vi "Lock-in_dem_mul Multiple Inputs and Outputs.vi"(3 "Phase&Tc":T1(array[cluster])=[{"Phase"=-4.587448254233148, "Time constant"=0.10000000000000009, "Set TimeConstant"=FALSE, "Autophase"=FALSE, "Order"=2.0}, {"Phase"=0.0, "Time constant"=0.2, "Set TimeConstant"=FALSE, "Autophase"=FALSE, "Order"=2.0}, {"Phase"=0.0, "Time constant"=0.0, "Set TimeConstant"=FALSE, "Autophase"=FALSE, "Order"=0.0}, {"Phase"=0.0, "Time constant"=0.0, "Set TimeConstant"=FALSE, "Autophase"=FALSE, "Order"=0.0}] {"Phase" min=0.0 max=360.0 scale=0.0..360.0}, 4 "Ref in":T2(array[cluster])=[{"Ref X"=array[40000 elements], "Ref Y"=array[40000 elements], "AI Rate"=200000.0, "AI Block Size"=40000.0, "Frequency"=20.0, "Ref amp"=5.0}, {"Ref X"=array[40000 elements], "Ref Y"=array[40000 elements], "AI Rate"=200000.0, "AI Block Size"=40000.0, "Frequency"=20.0, "Ref amp"=5.0}, {"Ref X"=array[40000 elements], "Ref Y"=array[40000 elements], "AI Rate"=200000.0, "AI Block Size"=40000.0, "Frequency"=20.0, "Ref amp"=5.0}, {"Ref X"=array[40000 elements], "Ref Y"=array[40000 elements], "AI Rate"=200000.0, "AI Block Size"=40000.0, "Frequency"=20.0, "Ref amp"=5.0}] {"Ref amp" step=0.001 format="%0.4f"; "Frequency" step=0.001 format="%0.4f"; "AI Block Size" step=0.001 format="%0.4f"; "AI Rate" step=0.001 format="%0.4f"}, 5 "Signal":dbl[][](array[numeric])=array4x40000[160000 elements]) -> (1 "Demodulation":dbl[][](array[numeric])=[[0.032308985716257205, -0.0020089800684537727, 0.032371384878394444, -3.5583001590229886], [0.023385861272623584, -0.0014539178662531169, 0.02343101330770514, -3.5574201885889787], [-3.111140914765216e-05, 2.7289487058700542e-06, 3.123206852318323e-05, -5.0131650508604935], [-3.1370210865590166e-05, 3.1631661467659442e-06, 3.1532606636697875e-05, -5.751181571584788]])   [LabVIEW 2013]
uses:
  <vilib>/Analysis/3filter.llb/Filter Passband Type.ctl
  <vilib>/Analysis/baseanly.llb/Mean (DBL).vi
  <vilib>/ptbypt/NI_PtbyPt.lvlib
  <vilib>/Analysis/NI_AALBase.lvlib
panel:
  out "Waveform Chart":dbl[][](graph)
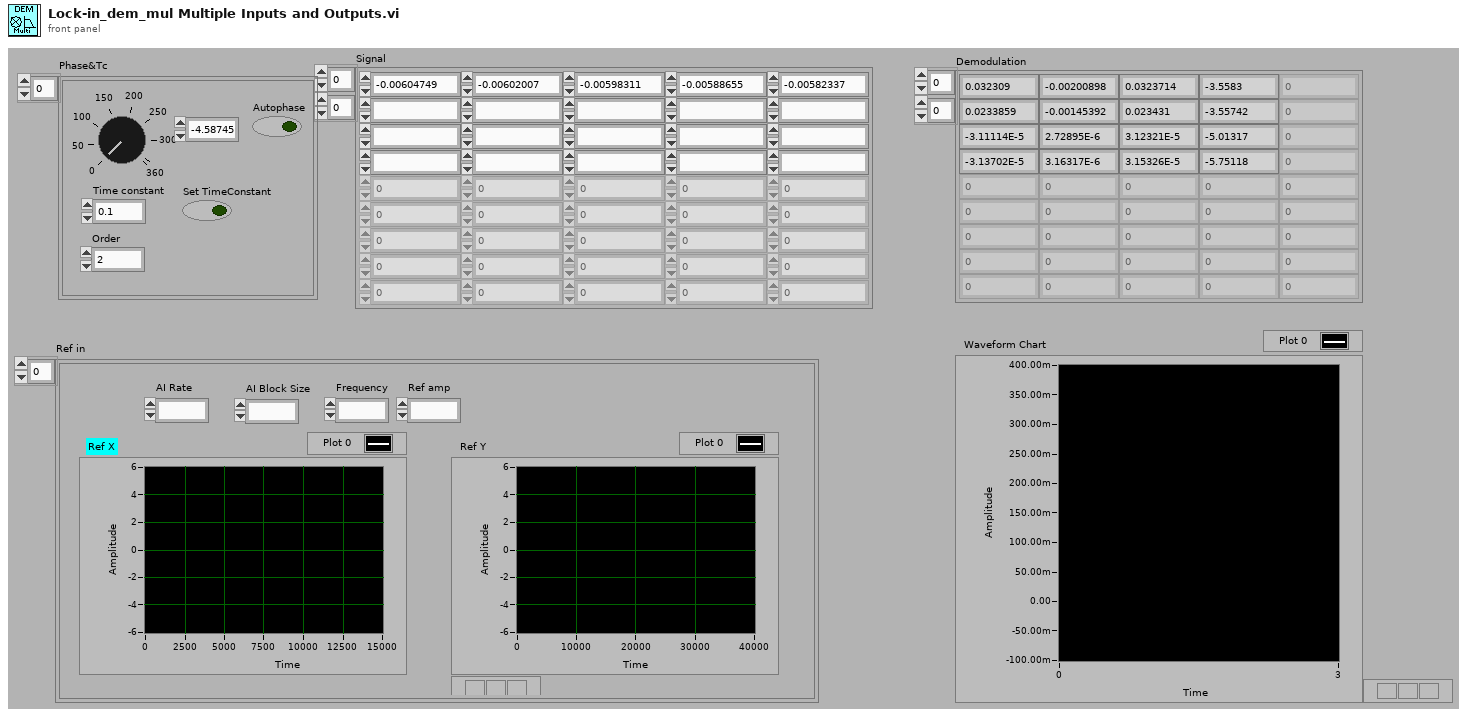
[diagram p1: front panel]
types:
  T1 = cluster{"Phase":dbl, "Time constant":dbl, "Set TimeConstant":bool, "Autophase":bool, "Order":dbl}[]
  T2 = cluster{"Ref X":dbl[], "Ref Y":dbl[], "AI Rate":dbl, "AI Block Size":dbl, "Frequency":dbl, "Ref amp":dbl}[]
  T3 = typedef "NI_AALBase.lvlib/Filter Passband Type.ctl" = enum32{"Lowpass", "Highpass", "Bandpass", "Bandstop"}
  T4 = cluster{"Ref X":dbl[], "Ref Y":dbl[], "AI Rate":dbl, "AI Block Size":dbl, "Frequency":dbl, "Ref amp":dbl}
  T5 = cluster{"Phase":dbl, "Time constant":dbl, "Set TimeConstant":bool, "Autophase":bool, "Order":dbl}
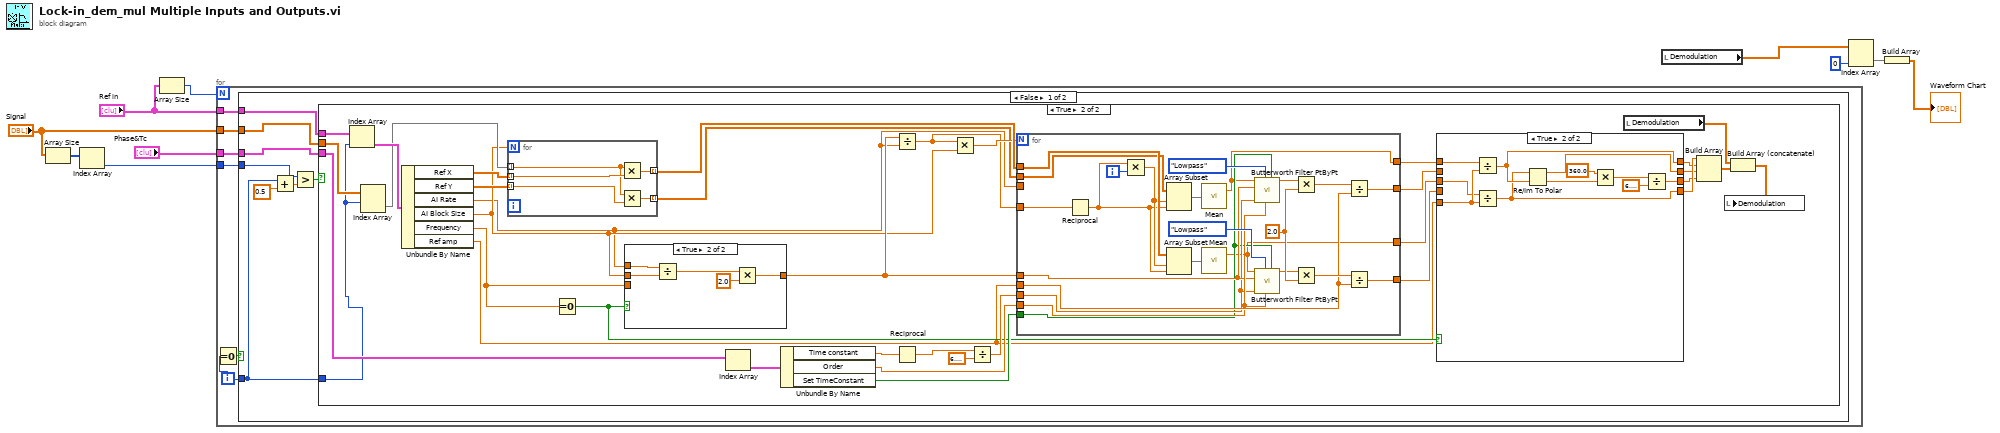
[diagram p0: block diagram]
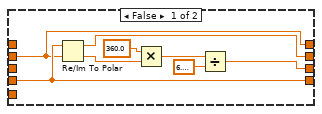
[diagram p3: hidden frame]
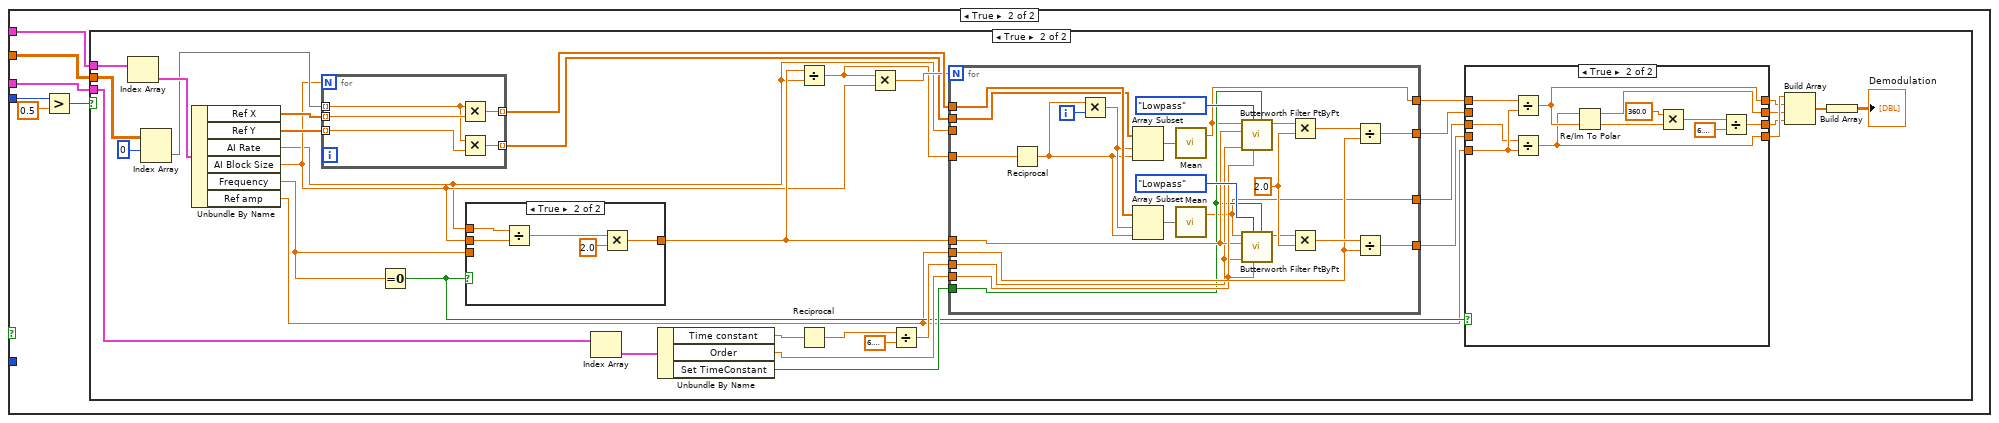
[diagram p5: hidden frame]
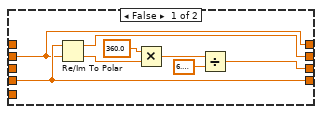
[diagram p7: hidden frame]
diagram:
  n1 = Array Size(array="Signal") -> (size(s)=w10:i32[])
  n2 = Index Array(array=w10) -> (element=w7:i32)  [unwired: 1 in]
  n3 = Array Size(array="Ref in") -> (size(s)=w5:i32)
  n4 = for {
    N: w5 -> [_]
    tunnel: "Ref in" -> [w16]
    tunnel: "Signal" -> [w15]
    tunnel: "Phase&Tc" -> [w14]
    tunnel: w7 -> [w13]
    i -> [w12]
    n5 = Equal To 0?(x=w12) -> (x = 0?=w11:bool)
    n6 = case shown="False" w11 {
      tunnel: w16 -> [w23 w118]
      tunnel: w15 -> [w22 w117]
      tunnel: w14 -> [w21 w116]
      tunnel: w13 -> [w18 w115]
      tunnel: w12 -> [w17 _]
      frame False {
        n7 = Add(x=w17, y=0.5) -> (x+y=w20:dbl)
        n8 = Greater?(x=w18, y=w20) -> (0:w24:bool)
        n9 = case shown="True" w24 {
          tunnel: w22 -> [_ w49]
          tunnel: w23 -> [_ w48]
          tunnel: w21 -> [_ w46]
          tunnel: w17 -> [_ w25]
          frame False {
          }
          frame True {
            n10 = Index Array(array=w48, index=w25) -> (element=w47:T4)
            n11 = Index Array(array=w49, index (row)=w25) -> (element=w43:dbl[])  [unwired: 1 in]
            n12 = Unbundle By Name(w47) -> ("Ref X"=w53:dbl[], "Ref Y"=w52:dbl[], "AI Rate"=w39:dbl, "AI Block Size"=w40:dbl, "Frequency"=w42:dbl, "Ref amp"=w28:dbl)
            n13 = for {
              N: w40 -> [_]
              tunnel: w43 -> [w112] mode=indexing
              tunnel: w53 -> [w114] mode=indexing
              tunnel: [w113] -> w60 mode=indexing
              tunnel: w52 -> [w111] mode=indexing
              tunnel: [w110] -> w57 mode=indexing
              n14 = Multiply(x=w112, y=w114) -> (x*y=w113:dbl)
              n15 = Multiply(x=w112, y=w111) -> (x*y=w110:dbl)
            }
            n16 = Equal To 0?(x=w42) -> (x = 0?=w38:bool)
            n17 = case shown="True" w38 {
              tunnel: w42 -> [w80 _]
              tunnel: [w80 w81] -> w41
              tunnel: w40 -> [_ w85]
              tunnel: w39 -> [_ w84]
              frame False {
              }
              frame True {
                n18 = Divide(x=w84, y=w85) -> (x/y=w83:dbl)
                n19 = Multiply(x=w83, y=2.0) -> (x*y=w81:dbl)
              }
            }
            n20 = Index Array(array=w46) -> (element=w45:T5)  [unwired: 1 in]
            n21 = Unbundle By Name(w45) -> ("Time constant"=w51:dbl, "Order"=w50:dbl, "Set TimeConstant"=w44:bool)
            n22 = Divide(x=w41, y=w39) -> (x/y=w58:dbl)
            n23 = Reciprocal(x=w51) -> (1/x=w56:dbl)
            n24 = Multiply(x=w58, y=w40) -> (x*y=w59:dbl)
            n25 = Divide(x=w56, y=6.283185307179586) -> (x/y=w54:dbl)
            n26 = for {
              N: w59 -> [_]
              tunnel: w39 -> [_]
              tunnel: w60 -> [w109]
              tunnel: w58 -> [w102]
              tunnel: w57 -> [w107]
              tunnel: w54 -> [w92]
              tunnel: w28 -> [w95]
              tunnel: w50 -> [w94]
              tunnel: w41 -> [w93]
              tunnel: w44 -> [w91]
              tunnel: [w89] -> w37
              tunnel: [w88] -> w36
              tunnel: [w87] -> w35
              tunnel: [w86] -> w34
              i -> [w108]
              w97 = 2.0 ("y")
              n27 = Reciprocal(x=w102) -> (1/x=w105:dbl)
              n28 = Multiply(x=w105, y=w108) -> (x*y=w106:dbl)
              n29 = Array Subset(array=w107, index=w106, length=w105) -> (w103:dbl[])
              n30 = Array Subset(array=w109, index=w106, length=w105) -> (w104:dbl[])
              n31 = call-poly <vilib>:"Mean.vi"("X"=w103) -> ("mean"=w86:dbl)  [unwired: 1 out]
              n32 = call-poly <vilib>:"Mean.vi"("X"=w104) -> ("mean"=w87:dbl)  [unwired: 1 out]
              n33 = call <vilib>:"Butterworth Filter PtByPt.vi"("initialize"=w91, "order"=w94, "filter type"=Filter_Passband_Type."Lowpass", "low cutoff freq: fl"=w92, "sampling freq: fs"=w93, "x"=w86) -> ("Filtered x"=w98:dbl)  [unwired: 3 in, 1 out]
              n34 = call <vilib>:"Butterworth Filter PtByPt.vi"("initialize"=w91, "order"=w94, "filter type"=Filter_Passband_Type."Lowpass", "low cutoff freq: fl"=w92, "sampling freq: fs"=w93, "x"=w87) -> ("Filtered x"=w90:dbl)  [unwired: 3 in, 1 out]
              n35 = Multiply(x=w98, y=w97) -> (x*y=w96:dbl)
              n36 = Multiply(x=w90, y=w97) -> (x*y=w99:dbl)
              n37 = Divide(x=w96, y=w95) -> (x/y=w88:dbl)
              n38 = Divide(x=w99, y=w95) -> (x/y=w89:dbl)
            }
            n39 = case shown="True" w38 {
              tunnel: w37 -> [w64 _]
              tunnel: w36 -> [w63 _]
              tunnel: w35 -> [_ w72]
              tunnel: w34 -> [_ w73]
              tunnel: [w64 w70] -> w33
              tunnel: [w63 w71] -> w32
              tunnel: [w62 w76] -> w31
              tunnel: [w61 w69] -> w30
              tunnel: w28 -> [_ w74]
              frame False {
                n40 = Re/Im To Polar(2:w63, 3:w64) -> (0:w68:dbl, 1:w62:dbl)
                n41 = Multiply(x=360.0 ("y"), y=w68) -> (x*y=w65:dbl)
                n42 = Divide(x=w65, y=6.283185307179586) -> (x/y=w61:dbl)
              }
              frame True {
                n43 = Divide(x=w73, y=w74) -> (x/y=w71:dbl)
                n44 = Divide(x=w72, y=w74) -> (x/y=w70:dbl)
                n45 = Re/Im To Polar(2:w71, 3:w70) -> (0:w75:dbl, 1:w76:dbl)
                n46 = Multiply(x=360.0 ("y"), y=w75) -> (x*y=w77:dbl)
                n47 = Divide(x=w77, y=6.283185307179586) -> (x/y=w69:dbl)
              }
            }
            n48 = local read "Demodulation"() -> (w27:dbl[][])
            n49 = Build Array(w33, w32, w31, w30) -> (w29:dbl[])
            n50 = Build Array (concatenate)(w27, w29) -> (w26:dbl[][])
            n51 = local write "Demodulation"(w26) -> ()
          }
        }
      }
      frame True {
        n52 = Greater?(x=w115, y=0.5) -> (0:w119:bool)
        n53 = case shown="True" w119 {
          tunnel: w117 -> [_ w144]
          tunnel: w118 -> [_ w143]
          tunnel: w116 -> [_ w122]
          frame False {
          }
          frame True {
            n54 = Index Array(array=w143) -> (element=w142:T4)  [unwired: 1 in]
            n55 = Index Array(array=w144, index (row)=0) -> (element=w139:dbl[])  [unwired: 1 in]
            n56 = Unbundle By Name(w142) -> ("Ref X"=w148:dbl[], "Ref Y"=w147:dbl[], "AI Rate"=w135:dbl, "AI Block Size"=w136:dbl, "Frequency"=w138:dbl, "Ref amp"=w123:dbl)
            n57 = for {
              N: w136 -> [_]
              tunnel: w139 -> [w207] mode=indexing
              tunnel: w148 -> [w209] mode=indexing
              tunnel: [w208] -> w155 mode=indexing
              tunnel: w147 -> [w206] mode=indexing
              tunnel: [w205] -> w152 mode=indexing
              n58 = Multiply(x=w207, y=w209) -> (x*y=w208:dbl)
              n59 = Multiply(x=w207, y=w206) -> (x*y=w205:dbl)
            }
            n60 = Equal To 0?(x=w138) -> (x = 0?=w134:bool)
            n61 = case shown="True" w134 {
              tunnel: w138 -> [w175 _]
              tunnel: [w175 w176] -> w137
              tunnel: w136 -> [_ w180]
              tunnel: w135 -> [_ w179]
              frame False {
              }
              frame True {
                n62 = Divide(x=w179, y=w180) -> (x/y=w178:dbl)
                n63 = Multiply(x=w178, y=2.0) -> (x*y=w176:dbl)
              }
            }
            n64 = Index Array(array=w122) -> (element=w141:T5)  [unwired: 1 in]
            n65 = Unbundle By Name(w141) -> ("Time constant"=w146:dbl, "Order"=w145:dbl, "Set TimeConstant"=w140:bool)
            n66 = Divide(x=w137, y=w135) -> (x/y=w153:dbl)
            n67 = Reciprocal(x=w146) -> (1/x=w151:dbl)
            n68 = Multiply(x=w153, y=w136) -> (x*y=w154:dbl)
            n69 = Divide(x=w151, y=6.283185307179586) -> (x/y=w149:dbl)
            n70 = for {
              N: w154 -> [_]
              tunnel: w135 -> [_]
              tunnel: w155 -> [w204]
              tunnel: w153 -> [w197]
              tunnel: w152 -> [w202]
              tunnel: w149 -> [w187]
              tunnel: w123 -> [w190]
              tunnel: w145 -> [w189]
              tunnel: w137 -> [w188]
              tunnel: w140 -> [w186]
              tunnel: [w184] -> w133
              tunnel: [w183] -> w132
              tunnel: [w182] -> w131
              tunnel: [w181] -> w130
              i -> [w203]
              w192 = 2.0 ("y")
              n71 = Reciprocal(x=w197) -> (1/x=w200:dbl)
              n72 = Multiply(x=w200, y=w203) -> (x*y=w201:dbl)
              n73 = Array Subset(array=w202, index=w201, length=w200) -> (w198:dbl[])
              n74 = Array Subset(array=w204, index=w201, length=w200) -> (w199:dbl[])
              n75 = call-poly <vilib>:"Mean.vi"("X"=w198) -> ("mean"=w181:dbl)  [unwired: 1 out]
              n76 = call-poly <vilib>:"Mean.vi"("X"=w199) -> ("mean"=w182:dbl)  [unwired: 1 out]
              n77 = call <vilib>:"Butterworth Filter PtByPt.vi"("initialize"=w186, "order"=w189, "filter type"=Filter_Passband_Type."Lowpass", "low cutoff freq: fl"=w187, "sampling freq: fs"=w188, "x"=w181) -> ("Filtered x"=w193:dbl)  [unwired: 3 in, 1 out]
              n78 = call <vilib>:"Butterworth Filter PtByPt.vi"("initialize"=w186, "order"=w189, "filter type"=Filter_Passband_Type."Lowpass", "low cutoff freq: fl"=w187, "sampling freq: fs"=w188, "x"=w182) -> ("Filtered x"=w185:dbl)  [unwired: 3 in, 1 out]
              n79 = Multiply(x=w193, y=w192) -> (x*y=w191:dbl)
              n80 = Multiply(x=w185, y=w192) -> (x*y=w194:dbl)
              n81 = Divide(x=w191, y=w190) -> (x/y=w183:dbl)
              n82 = Divide(x=w194, y=w190) -> (x/y=w184:dbl)
            }
            n83 = case shown="True" w134 {
              tunnel: w133 -> [w159 _]
              tunnel: w132 -> [w158 _]
              tunnel: w131 -> [_ w167]
              tunnel: w130 -> [_ w168]
              tunnel: [w159 w165] -> w129
              tunnel: [w158 w166] -> w128
              tunnel: [w157 w171] -> w127
              tunnel: [w156 w164] -> w126
              tunnel: w123 -> [_ w169]
              frame False {
                n84 = Re/Im To Polar(2:w158, 3:w159) -> (0:w163:dbl, 1:w157:dbl)
                n85 = Multiply(x=360.0 ("y"), y=w163) -> (x*y=w160:dbl)
                n86 = Divide(x=w160, y=6.283185307179586) -> (x/y=w156:dbl)
              }
              frame True {
                n87 = Divide(x=w168, y=w169) -> (x/y=w166:dbl)
                n88 = Divide(x=w167, y=w169) -> (x/y=w165:dbl)
                n89 = Re/Im To Polar(2:w166, 3:w165) -> (0:w170:dbl, 1:w171:dbl)
                n90 = Multiply(x=360.0 ("y"), y=w170) -> (x*y=w172:dbl)
                n91 = Divide(x=w172, y=6.283185307179586) -> (x/y=w164:dbl)
              }
            }
            n92 = Build Array(w129, w128, w127, w126) -> (w125:dbl[])
            n93 = Build Array(w125) -> (→"Demodulation":dbl[][])
          }
        }
      }
    }
  }
  n94 = local read "Demodulation"() -> (w4:dbl[][])
  n95 = Index Array(array=w4, index (col)=0 ("disabled index (col)")) -> (element=w3:dbl[])  [unwired: 1 in]
  n96 = Build Array(w3) -> (→"Waveform Chart":dbl[][])
